vi "Open Connection.vi"(8 "error in (no error)":errorcluster, 11 "Device":string="hidraw0") -> (0 "error out":errorcluster, 3 "HID Handle":i64)   [LabVIEW 2021, in "USB Relay Control.lvlib"]
uses:
  USB Relay Control.lvlib
  typedef/Errors.ctl
  Add USB Relay Error Core.vi
  kernel32.dll
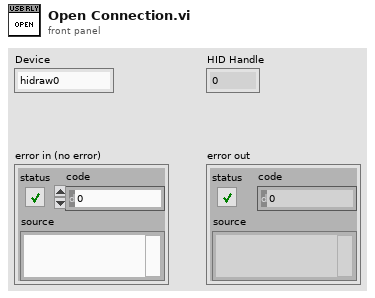
[diagram p1: front panel]
types:
  T1 = typedef "USB Relay Control.lvlib/Errors.ctl" = enum16{"Invalid ID", "Failed to write ID", "Invalid Device"}
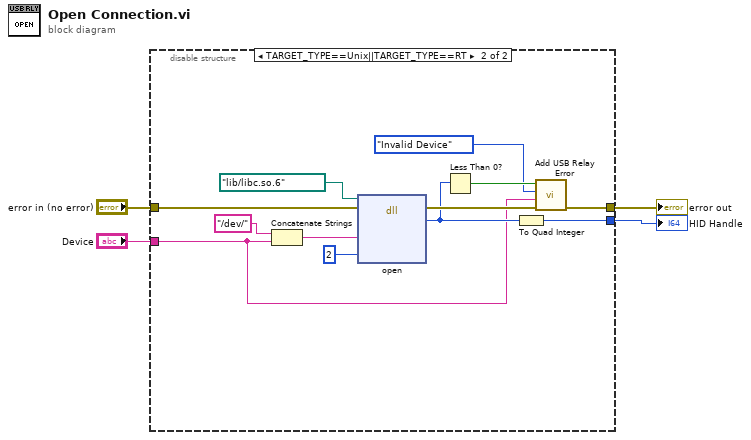
[diagram p0: block diagram]
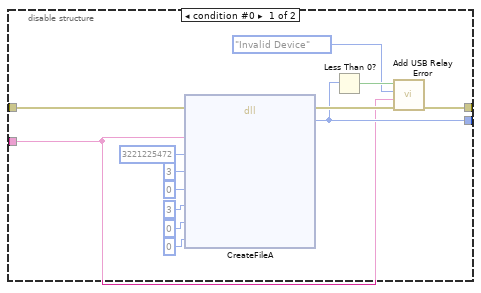
[diagram p2: hidden frame]
diagram:
  n1 = disable-structure shown="TARGET_TYPE==Unix||TARGET_TYPE==RT" {
    disable-tunnel: "error in (no error)" -> [w17 w28]
    disable-tunnel: [w15 w23] -> w3
    disable-tunnel: "Device" -> [w5 w19]
    disable-tunnel: [w12 w18] -> w1
    frame condition #0 {
      n2 = dll-call lib="kernel32.dll" fn="CreateFileA"(error in=w17, "lpFileName"=w5, "dwDesiredAccess"=u32 3221225472, "dwShareMode"=u32 3, "lpSecurityAttributes"=u64 0, "dwCreationDisposition"=u32 3, "dwFlagsAndAttributes"=u32 0, "hTemplateFile"=u64 0) -> (error out=w16:errorcluster, "return type"=w12:i64)  [unwired: 9 in, 1 out]
      n3 = Less Than 0?(x=w12) -> (x < 0?=w14:bool)
      n4 = call "Add USB Relay Error.vi"("error in (no error)"=w16, "String to Append"=w5, "Error"=Errors."Invalid Device", "Insert Error"=w14) -> ("error out"=w15:errorcluster)  [unwired: 7 in]
    }
    frame condition #1 (active) {
      n5 = Concatenate Strings("/dev/" ("path"), w19) -> (w25:string)
      n6 = dll-call lib="lib/librt.so.1" fn="open"(path in=path "/lib/libc.so.6" ("librt path"), error in=w28, "path"=w25, "flags"=2) -> (error out=w24:errorcluster, "return type"=w21:i32)  [unwired: 3 in, 1 out]
      n7 = Less Than 0?(x=w21) -> (x < 0?=w22:bool)
      n8 = To Quad Integer(1:w21) -> (0:w18:i64)
      n9 = call "Add USB Relay Error.vi"("error in (no error)"=w24, "String to Append"=w19, "Error"=Errors."Invalid Device", "Insert Error"=w22) -> ("error out"=w23:errorcluster)  [unwired: 7 in]
    }
  }
  "error out" <- w3
  "HID Handle" <- w1
